vi "Web Root.vi"() -> (7 "WWW Root":path)   [LabVIEW 2020, in "Volatus.lvlib" / "Volatus Core.lvclass"]
uses:
  Volatus Core.lvclass
  Volatus Core.lvclass/Volatus Core.ctl
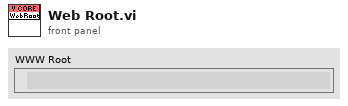
[diagram p1: front panel]
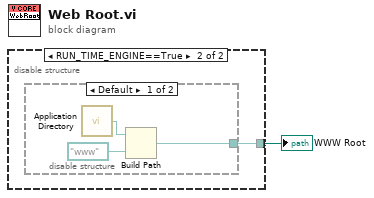
[diagram p0: block diagram]
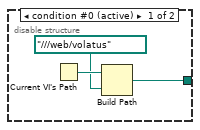
[diagram p2: hidden frame]
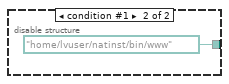
[diagram p3: hidden frame]
diagram:
  n1 = disable-structure shown="RUN_TIME_ENGINE==True" {
    disable-tunnel: [w2 w5] -> w1
    frame condition #0 (active) {
      n2 = Current VI's Path() -> (path=w4:path)
      n3 = Build Path(base path=w4, name or relative path=path "../../../web/volatus") -> (appended path=w2:path)
    }
    frame condition #1 {
      n4 = disable-structure shown="Default" {
        disable-tunnel: [w6 path "home/lvuser/natinst/bin/www" ("appended path")] -> w5
        frame condition #0 (active) {
          n5 = call <vilib>:"Application Directory.vi"() -> ("Application Directory"=w8:path)
          n6 = Build Path(base path=w8, name or relative path=path "www") -> (appended path=w6:path)
        }
        frame condition #1 {
        }
      }
    }
  }
  "WWW Root" <- w1
